vi "Calculate CRC32.vi"(8 "error in":errorcluster, 11 "data bytes":u8[](array[numeric])) -> (0 "error out":errorcluster, 3 "crc32":u32)   [LabVIEW 2015, in "Lengmur_socket.lvlib"]
uses:
  Lengmur_socket.lvlib
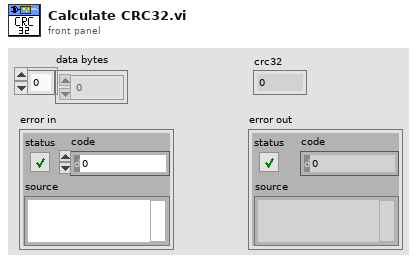
[diagram p1: front panel]
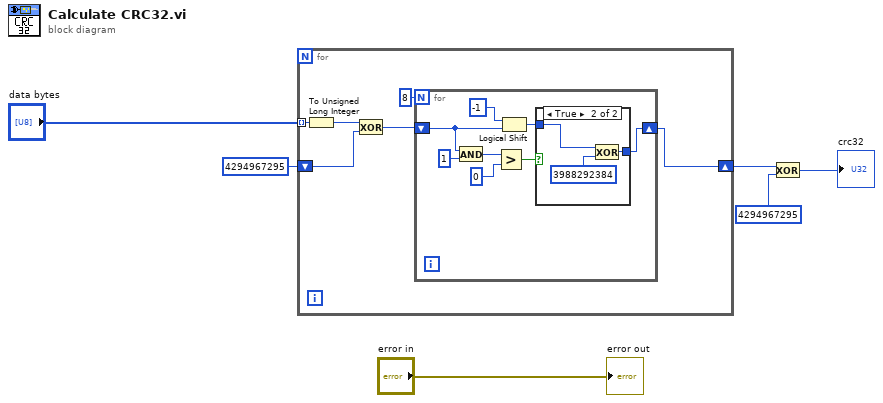
[diagram p0: block diagram]
diagram:
  n1 = for {
    tunnel: "data bytes" -> [w12] mode=indexing
    shift-right: [w8] -> w4
    shift-left: u32 4294967295 -> [w9]
    n2 = To Unsigned Long Integer(number=w12) -> (unsigned 32bit integer=w10:u32)
    n3 = Exclusive Or(1:w9, 2:w10) -> (0:w7:u32)
    n4 = for {
      N: 8 -> [_]
      shift-right: [w14] -> w8
      shift-left: w7 -> [w13]
      n5 = And(x=w13, y=u32 1) -> (x .and. y?=w18:u32)
      n6 = Greater?(x=w18, y=u32 0) -> (0:w16:bool)
      n7 = Logical Shift(y=i16 -1, x=w13) -> (x << y=w15:u32)
      n8 = case shown="True" w16 {
        tunnel: w15 -> [w21 w22]
        tunnel: [w21 w23] -> w14
        frame False {
        }
        frame True {
          n9 = Exclusive Or(1:u32 3988292384 ("y"), 2:w22) -> (0:w23:u32)
        }
      }
    }
  }
  n10 = Exclusive Or(1:u32 4294967295, 2:w4) -> (0:→"crc32":u32)
  "error out" <- "error in"
